vi "Demo - blink.vi"() -> ()   [LabVIEW 2021]
uses:
  LED typedef.ctl
panel:
  out "error out":errorcluster
  in  "LED":T1
  in  "port":u32
  in  "Base URL":string
  in  "stop":bool
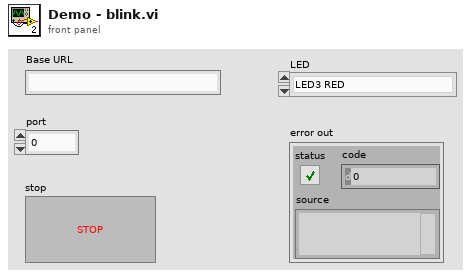
[diagram p1: front panel]
types:
  T1 = typedef "LED typedef.ctl" = enum16{"LED3 RED", "LED3 GREEN", "LED3 BLUE", "LED4 RED", "LED4 GREEN", "LED4 BLUE"}
  T2 = typedef "UNO Q Session.ctl" = cluster{"HTTP client":T3, "Base URL":string, "Connected":bool}
  T3 = typedef "LabVIEWHTTPClient.lvlib/ClientHandle.ctl" = refnum<k1>
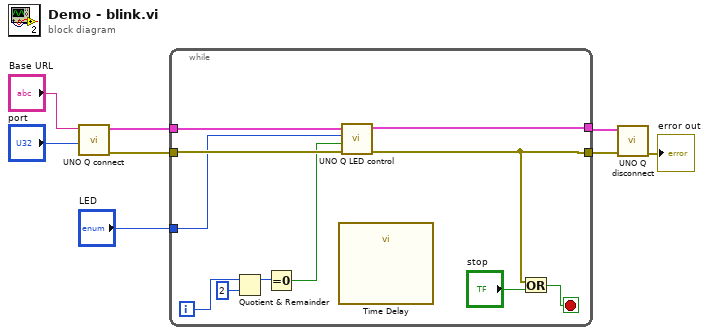
[diagram p0: block diagram]
diagram:
  n1 = call "UNO Q connect.vi"("port"="port", "Base URL"="Base URL") -> ("error out"=w5:errorcluster, "Session out"=w6:T2)  [unwired: 4 in]
  n2 = while {
    tunnel: w6 -> [w15]
    tunnel: w5 -> [w16]
    tunnel: "LED" -> [w14]
    tunnel: [w12] -> w3
    tunnel: [w9] -> w2
    i -> [w19]
    stop <- w10 stop-if-true
    n3 = Quotient & Remainder(x=w19, y=2) -> (x-y*floor(x/y)=w17:i32)  [unwired: 1 out]
    n4 = Equal To 0?(x=w17) -> (x = 0?=w13:bool)
    n5 = call "Time Delay"() -> ()  [unwired: 11 in, 1 out]
    n6 = call "UNO Q LED control.vi"("error in (no error)"=w16, "State"=w13, "LED"=w14, "UNO Q Session in"=w15) -> ("error out"=w9:errorcluster, "UNO Q Session out"=w12:T2)  [unwired: 4 in, 2 out]
    n7 = Or(x=w9, y="stop") -> (x .or. y?=w10:bool)
  }
  n8 = call "UNO Q disconnect.vi"("error in (no error)"=w2, "UNO Q Session"=w3) -> ("error out"=→"error out":errorcluster)  [unwired: 9 in]
